vi "Pre Launch Init.vi"(11 "Nested in":refnum<class "ChannelManagerUI.lvclass">) -> (0 "error out":errorcluster, 3 "Nested out":refnum<class "ChannelManagerUI.lvclass">)   [LabVIEW 2021, in "Channel.lvlib" / "ChannelManagerUI.lvlib" / "ChannelManagerUI.lvclass"]
doc: "(<B>Filename</B>: Actor Framework.lvlib:Actor.lvclass:Pre Launch Init.vi)\n\nDefines behavior that occurs after the Launch Nested Actor method is invoked but before the actor's Actor Core method begins running.\n\nBy default, this method does nothing. A descendant class may override it to define behavior."
uses:
  ChannelManagerUI.lvclass
  ChannelManagerUI.lvclass/ChannelManagerUI.ctl
  ChannelsManager/ChannelsManager/ChannelsManager.lvclass
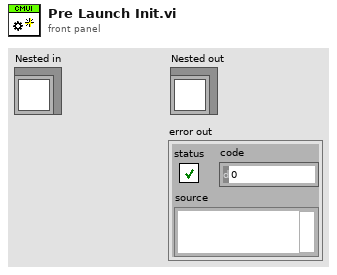
[diagram p1: front panel]
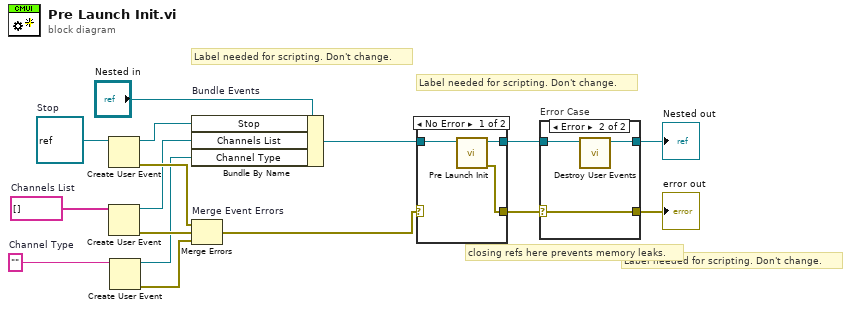
[diagram p0: block diagram]
diagram:
  w3 = ""  # Channel Type
  w6 = string[] []  # Channels List
  w8 = refnum<class> refnum  # Stop
  # "Label needed for scripting. Don't change."
  # "Label needed for scripting. Don't change."
  # "Label needed for scripting. Don't change."
  # "closing refs here prevents memory leaks."
  n1 = Create User Event(user event datatype=w8) -> (user event=w7:refnum<user-event>, error out=w15:errorcluster)  [unwired: 1 in]
  n2 = Create User Event(user event datatype=w6) -> (user event=w5:refnum<user-event>, error out=w4:errorcluster)  [unwired: 1 in]
  n3 = Create User Event(user event datatype=w3) -> (user event=w2:refnum<user-event>, error out=w1:errorcluster)  [unwired: 1 in]
  n4 = Bundle By Name "Bundle Events"(cluster="Nested in", "Stop"=w7, "Channels List"=w5, "Channel Type"=w2) -> (w11:refnum<class "ChannelManagerUI.lvclass">)
  n5 = Merge Errors "Merge Event Errors"(w15, w4, w1) -> (w10:errorcluster)
  n6 = case shown="No Error" w10 {
    selector: w10 -> [_ w21]
    tunnel: [w19 w20] -> w12
    tunnel: w11 -> [w18 w20]
    tunnel: [w17 w21] -> w9
    frame No Error {
      n7 = call-parent "Pre Launch Init.vi"("Actor in"=w18) -> ("error out"=w17:errorcluster, "Actor out"=w19:refnum<class "ChannelManagerUI.lvclass">)  [unwired: 9 in]
    }
    frame Error {
    }
  }
  n8 = case "Error Case" shown="Error" w9 {
    selector: w9 -> [w22 w26]
    tunnel: w12 -> [w23 w25]
    tunnel: [w23 w24] -> w14
    tunnel: [w22 w26] -> w13
    frame No Error {
    }
    frame Error {
      n9 = call "Destroy User Events.vi"("UI Template in"=w25) -> ("UI Template out"=w24:refnum<class "ChannelManagerUI.lvclass">)  [unwired: 10 in]
    }
  }
  "error out" <- w13
  "Nested out" <- w14
